vi "GetPanelUI.vi"(8 "error in (no error)":errorcluster, 11 "object in":refnum<class "AIO-Configuration.lvclass">) -> (0 "error out":errorcluster, 2 "VI Refnum":refnum<vi>, 3 "object out":refnum<class "AIO-Configuration.lvclass">)   [LabVIEW 2021, in "DAQmx.lvlib" / "AIO-Configuration.lvclass"]
uses:
  AIO-Configuration.lvclass
  AIO-DAQ-Panel.vi
  AIO-Configuration.lvclass/AIO-Configuration.ctl
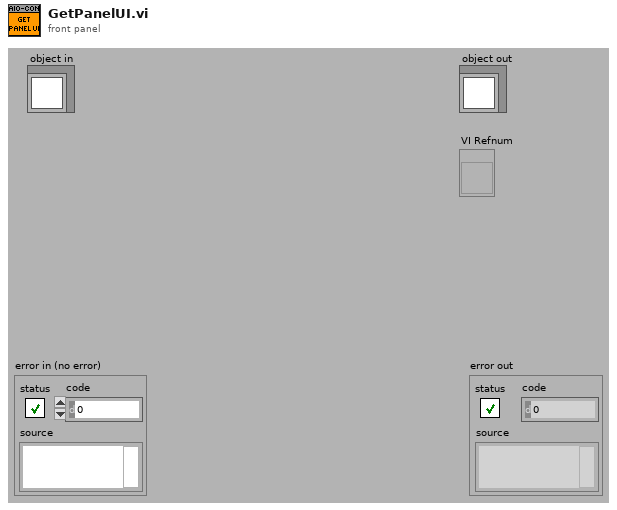
[diagram p1: front panel]
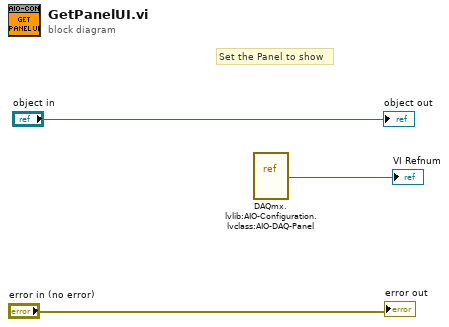
[diagram p0: block diagram]
diagram:
  # "Set the Panel to show"
  n1 = vi-ref "DAQmx.lvlib:AIO-Configuration.lvclass:AIO-DAQ-Panel.vi"() -> (→"VI Refnum":refnum<vi>)
  "error out" <- "error in (no error)"
  "object out" <- "object in"
